vi "SMTP Email Send Message Start.vi"(4 "error in (no error)":errorcluster caption="entrée d'erreur (pas d'erreur)", 5 "return address":string caption="adresse de retour", 6 "recipients":string[](array[string]) caption="destinataires", 7 "smtp session":T1 caption="session smtp") -> (0 "error out":errorcluster caption="sortie d'erreur", 2 "invalid recipients":string[](array[string]) caption="destinataires non valides", 3 "smtp session out":T1 caption="session smtp en sortie")   [LabVIEW 2022 SP3, in "Copie de NI_SMTPEmail.lvlib"]
uses:
  Copie de NI_SMTPEmail.lvlib
  SMTP Email Session.ctl
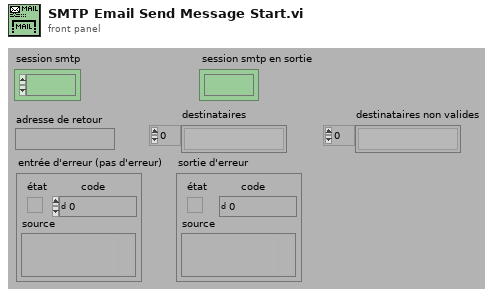
[diagram p1: front panel]
types:
  T1 = typedef "Copie de NI_SMTPEmail.lvlib/SMTP Email Session.ctl" = refnum<k1>
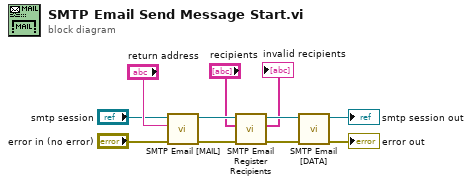
[diagram p0: block diagram]
diagram:
  n1 = call "SMTP Email [MAIL].vi"("error in (no error)"="error in (no error)", "return address"="return address", "smtp session"="smtp session") -> ("error out"=w9:errorcluster, "smtp session out"=w10:T1)  [unwired: 1 in, 2 out]
  n2 = call "SMTP Email Register Recipients.vi"("error in (no error)"=w9, "recipients"="recipients", "smtp session"=w10) -> ("error out"=w11:errorcluster, "invalid recipients"=→"invalid recipients":string[], "smtp session out"=w8:T1)  [unwired: 2 in]
  n3 = call "SMTP Email [DATA].vi"("error in (no error)"=w11, "smtp session"=w8) -> ("error out"=→"error out":errorcluster, "smtp session out"=→"smtp session out":T1)  [unwired: 2 in, 2 out]
